vi "Neuron_Selector.vi"(10 "Neuronal Model":T1(ring)) -> (0 "d":dbl, 1 "c":dbl, 2 "b":dbl, 3 "a":dbl, 4 "Model":string)   [LabVIEW 2025]
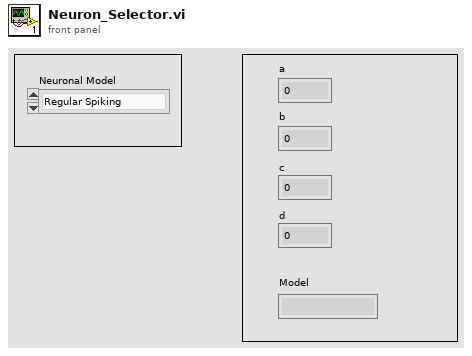
[diagram p1: front panel]
types:
  T1 = enum16{"Regular Spiking", "Chattering", "Fast Spiking"}
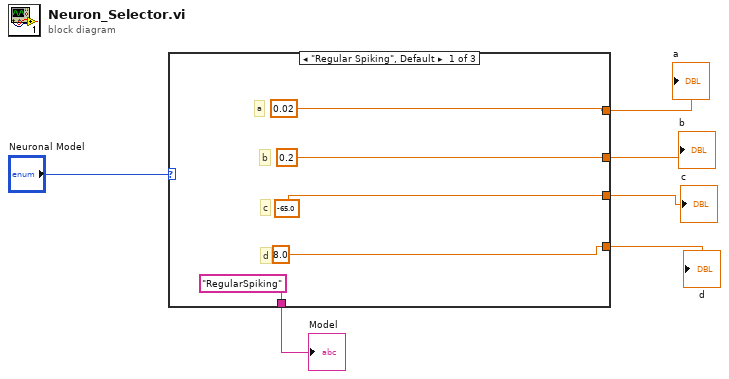
[diagram p0: block diagram]
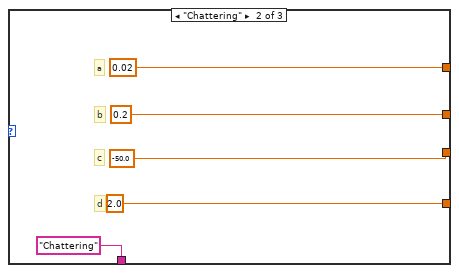
[diagram p2: hidden frame]
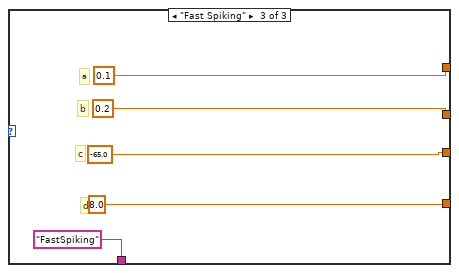
[diagram p3: hidden frame]
diagram:
  n1 = case shown="\"Regular Spiking\", Default" "Neuronal Model" {
    tunnel: [0.02 0.02 0.1] -> w5
    tunnel: [0.2 0.2 0.2] -> w4
    tunnel: [-65.0 -50.0 -65.0] -> w3
    tunnel: [8.0 2.0 8.0] -> w2
    tunnel: ["RegularSpiking" "Chattering" "FastSpiking"] -> w1
    frame "Regular Spiking", Default {
      # "d"
      # "c"
      # "b"
      # "a"
    }
    frame "Chattering" {
      # "d"
      # "c"
      # "b"
      # "a"
    }
    frame "Fast Spiking" {
      # "b"
      # "c"
      # "d"
      # "a"
    }
  }
  "a" <- w5
  "b" <- w4
  "c" <- w3
  "d" <- w2
  "Model" <- w1
